vi "XNET Signal Probe.vi"(0 "database":string="C:\\Users\\dihidalg\\Documents\\GIT\\Demos\\SnV-Flexlogger-Plugin-PoC\\src\\CAN\\eDyno_NVH_PoC.dbc", 5 "signals":string[](array[string])=["DYNO_Cmd.DynoCmd_Mode", "DYNO_Cmd.DynoCmd_Enable", "DYNO_Cmd.DynoCmd_Alive", "DYNO_Cmd.DynoCmd_SpeedSetpoint", "DYNO_Cmd.DynoCmd_RunUpStart", "DYNO_Cmd.DynoCmd_RunUpEnd", "DYNO_Cmd.DynoCmd_RunUpDuration", "DYNO_Cmd.DynoCmd_TestStep", "DYNO_Cmd.DynoCmd_TorqueSetpoint", "DYNO_Status.DynoSts_Mode", "DYNO_Status.DynoSts_AtSpeed", "DYNO_Status.DynoSts_SimRunning", "DYNO_Status.DynoSts_Alive", "DYNO_Status.DynoSts_SpeedAct", "DYNO_Status.DynoSts_TestStep", "DYNO_Status.DynoSts_BlockCounter", "DYNO_Status.DynoSts_TorqueAct", "SIM_FaultCmd.FltCmd_Imbalance_On", "SIM_FaultCmd.FltCmd_Misalign_On", "SIM_FaultCmd.FltCmd_BPFO_On", "SIM_FaultCmd.FltCmd_Ripple_On", "SIM_FaultCmd.FltCmd_PWM_On", "SIM_FaultCmd.FltCmd_Alive", "SIM_FaultCmd.FltCmd_Imbalance_Amp", "SIM_FaultCmd.FltCmd_Misalign_Amp", "SIM_FaultCmd.FltCmd_BPFO_Amp", "SIM_FaultCmd.FltCmd_Ripple_Amp", "SIM_FaultCmd.FltCmd_PWM_Amp", "SIM_FaultStatus.FltSts_Imbalance_On", "SIM_FaultStatus.FltSts_Misalign_On", "SIM_FaultStatus.FltSts_BPFO_On", "SIM_FaultStatus.FltSts_Ripple_On", "SIM_FaultStatus.FltSts_PWM_On", "SIM_FaultStatus.FltSts_ActiveId", "SIM_FaultStatus.FltSts_SeqState", "SIM_FaultStatus.FltSts_Alive", "SIM_FaultStatus.FltSts_Freq_1x", "SIM_FaultStatus.FltSts_Freq_2x", "SIM_FaultStatus.FltSts_Freq_BPFO", "SIM_FaultStatus.FltSts_Freq_Ripple", "SIM_FaultStatus.FltSts_Freq_PWM", "SIM_FaultStatus.FltSts_TestStep", "SIM_FaultStatus.FltSts_Imbalance_Amp", "SIM_FaultStatus.FltSts_Misalign_Amp", "SIM_FaultStatus.FltSts_BPFO_Amp", "SIM_FaultStatus.FltSts_Ripple_Amp", "SIM_FaultStatus.FltSts_PWM_Amp", "SIM_Config.SimCfg_BPFO_Order", "SIM_Config.SimCfg_Resonance", "SIM_Config.SimCfg_Decay", "SIM_Config.SimCfg_PolePairs", "SIM_Config.SimCfg_SampleRate", "SIM_Config.SimCfg_PWMCarrier", "SIM_Config.SimCfg_RefSpeed", "SIM_Config.SimCfg_Baseline1x", "SIM_Config.SimCfg_NoiseFloor"]) -> (4 "error codes":i32[](array[numeric]))   [LabVIEW 2026]
doc: "Opens a Conversion session per signal and reports the NI-XNET error code for each."
uses:
  <vilib>/xnet/xnet.llb/XNET Create Session (Generic).vi
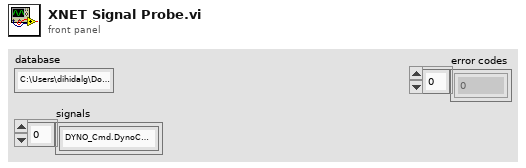
[diagram p1: front panel]
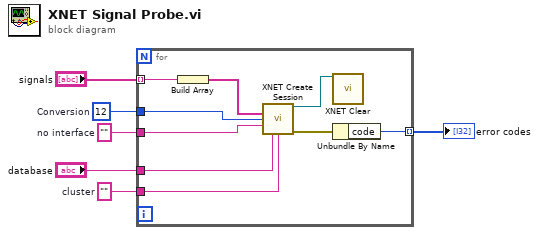
[diagram p0: block diagram]
diagram:
  w2 = ""  # cluster
  w3 = ""  # no interface
  w4 = u32 12  # Conversion
  n1 = for {
    tunnel: "signals" -> [w15] mode=indexing
    tunnel: "database" -> [w11]
    tunnel: w4 -> [w13]
    tunnel: w3 -> [w12]
    tunnel: w2 -> [w10]
    tunnel: [w7] -> w1 mode=indexing
    n2 = Build Array(w15) -> (w14:string[])
    n3 = call-poly <vilib>:"XNET Create Session.vi"("list (empty)"=w14, "mode"=w13, "interface"=w12, "database (:memory:)"=w11, "cluster (empty)"=w10) -> ("session out"=w8:refnum<k21>, "error out"=w9:errorcluster)  [unwired: 9 in]
    n4 = call <vilib>:"XNET Clear.vi"("session in"=w8) -> ()  [unwired: 14 in, 1 out]
    n5 = Unbundle By Name(w9) -> ("code"=w7:i32)
  }
  "error codes" <- w1
